vi "Data_Connect.vi"(8 "error in":errorcluster, 11 "IP myRIO in":string="172.22.11.2") -> (0 "error out":errorcluster, 1 "connected?":bool, 3 "reader endpoint out":refnum<k21>)   [LabVIEW 2025]
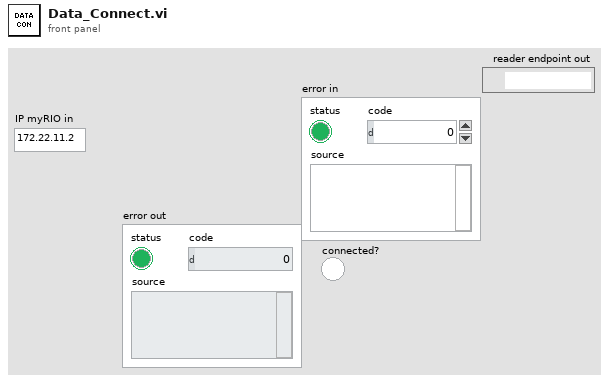
[diagram p1: front panel]
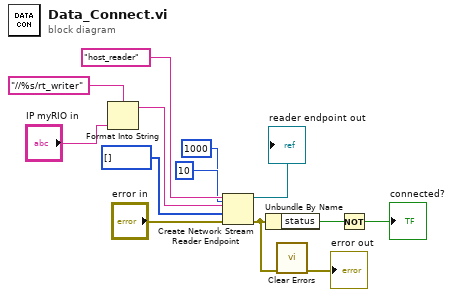
[diagram p0: block diagram]
diagram:
  n1 = Format Into String(format string="//%s/rt_writer", "IP myRIO in") -> (resulting string=w8:string)  [unwired: 2 in, 1 out]
  n2 = Create Network Stream Reader Endpoint(5:1000 ("timeout in ms (-1)"), 7:10 ("reader buffer size"), 8:"error in", 9:i16[] [], 10:w8, 11:"host_reader" ("writer name")) -> (0:w3:errorcluster, 3:→"reader endpoint out":refnum<k21>)  [unwired: 1 in]
  n3 = Unbundle By Name(w3) -> ("status"=w5:bool)
  n4 = call <vilib>:"Clear Errors.vi"("error in (no error)"=w3) -> ("error out"=→"error out":errorcluster)  [unwired: 5 in, 1 out]
  n5 = Not(x=w5) -> (.not. x?=→"connected?":bool)
